vi "C_CAN_Deserialize.vi"(8 "error in (no error)":errorcluster, 11 "payload":u8[](array[numeric]) format="%.0x") -> (0 "error out":errorcluster, 2 "decode errors":u32, 3 "frames":T1[](array[typedef]) {"id" format="%.0x"})   [LabVIEW 2021, in "CANsub_C.lvlib"]
doc: "Decodes all CAN frames of one HDLC payload from the CANsub into CAN_Frame clusters (device time, ID, flags, DLC, data). decode errors = 1 if the payload ended in a truncated frame. Allocates on every call: tests only."
uses:
  CANsub_C.lvlib
  common/Typedefs/Bytes.ctl
  common/CANsub_Common.lvlib
  common/Typedefs/CAN_Frame.ctl
  codec_vis/CANsub_Codec.lvlib
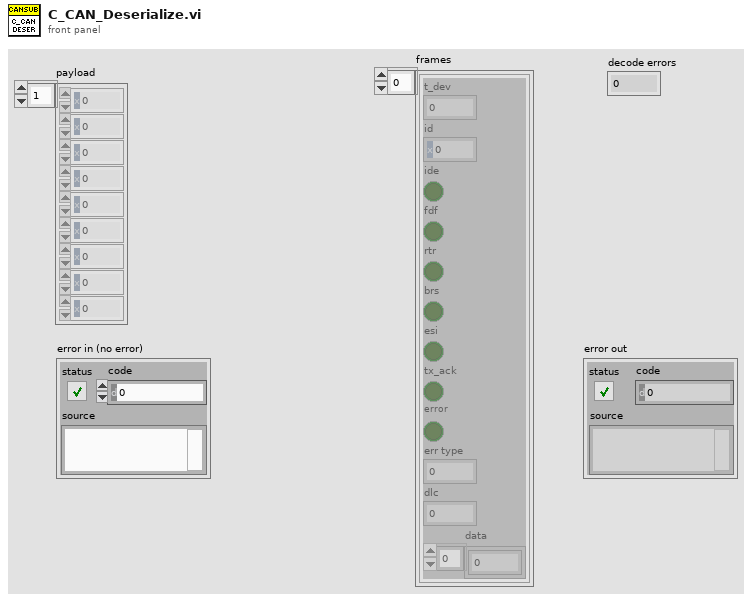
[diagram p1: front panel]
types:
  T1 = typedef "CANsub_Common.lvlib/CAN_Frame.ctl" = cluster{"t_dev":dbl, "id":u32, "ide":bool, "fdf":bool, "rtr":bool, "brs":bool, "esi":bool, "tx_ack":bool, "error":bool, "err type":u8, "dlc":u8, "data":T2}
  T2 = typedef "CANsub_Common.lvlib/Bytes.ctl" = u8[]
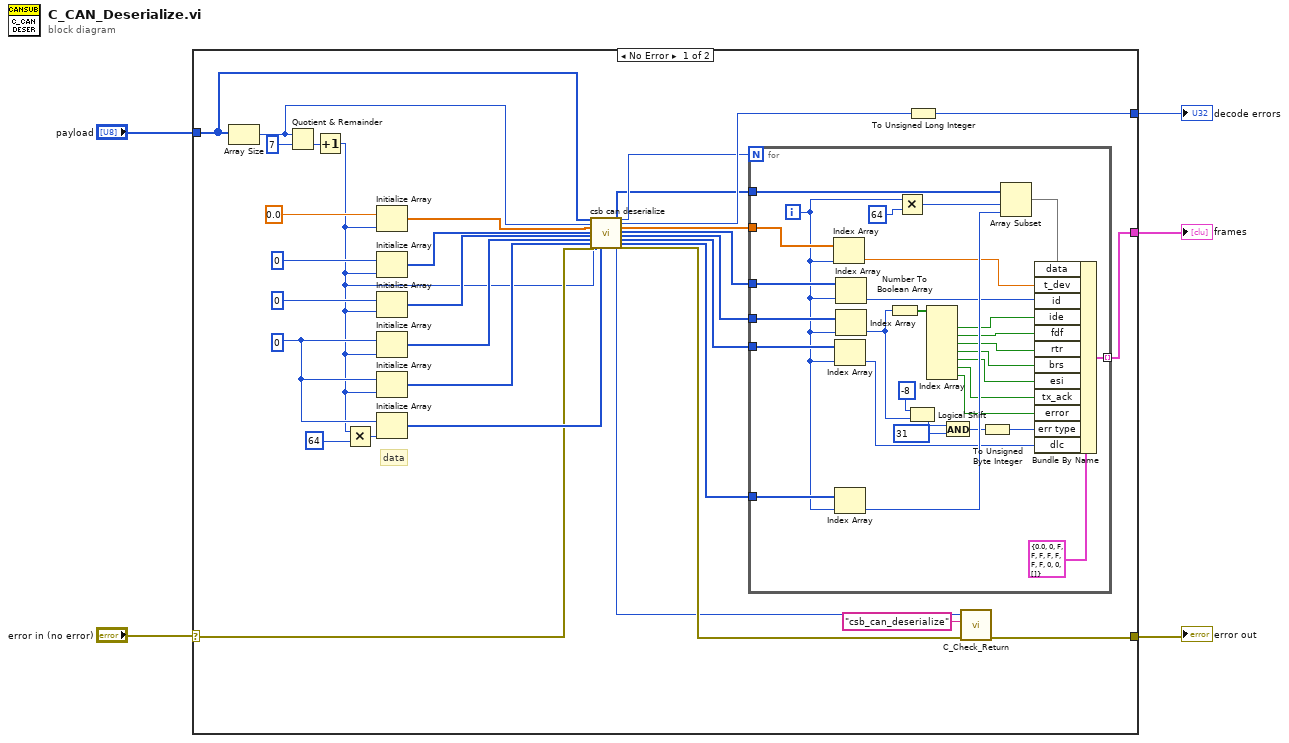
[diagram p0: block diagram]
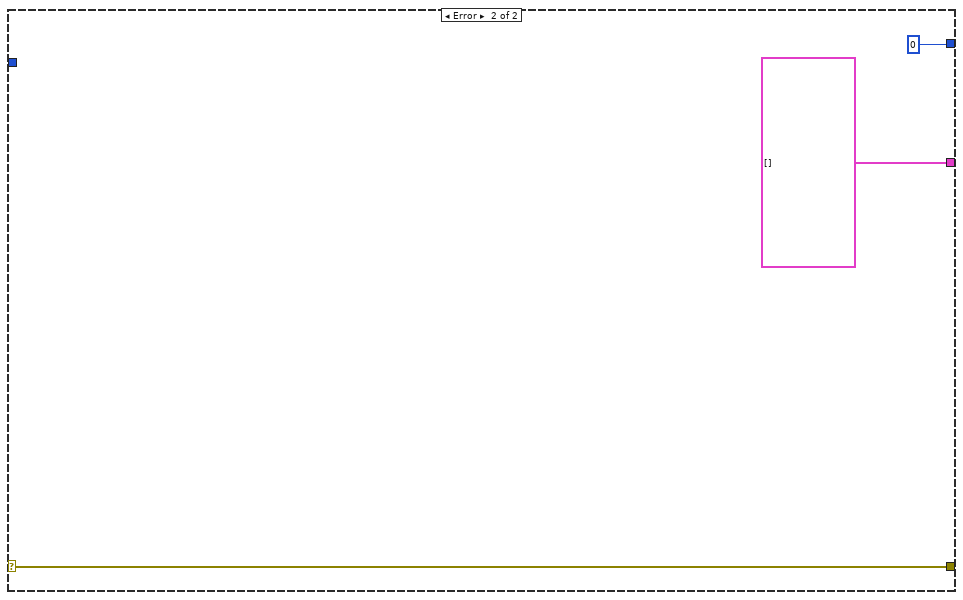
[diagram p2: hidden frame]
diagram:
  n1 = case shown="No Error" "error in (no error)" {
    selector: "error in (no error)" -> [w21 w70]
    tunnel: [w19 w70] -> w4
    tunnel: [w16 u32 0] -> w3
    tunnel: [w6 T1[] [] ("frames")] -> w2
    tunnel: "payload" -> [w28 _]
    frame No Error {
      w36 = u8 0
      # "data"
      n2 = Array Size(array=w28) -> (size(s)=w31:i32)
      n3 = Quotient & Remainder(x=w31, y=7) -> (floor(x/y)=w22:i32)  [unwired: 1 out]
      n4 = Increment(x=w22) -> (x+1=w18:i32)
      n5 = Multiply(x=w18, y=64) -> (x*y=w30:i32)
      n6 = Initialize Array(0.0, w18) -> (w32:dbl[])
      n7 = Initialize Array(u32 0, w18) -> (w23:u32[])
      n8 = Initialize Array(u16 0, w18) -> (w24:u16[])
      n9 = Initialize Array(w36, w18) -> (w25:u8[])
      n10 = Initialize Array(w36, w18) -> (w26:u8[])
      n11 = Initialize Array(w36, w30) -> (w27:u8[])
      n12 = call "csb can deserialize.vi"("payload"=w28, "len"=w31, "t_dev"=w32, "id"=w23, "flags"=w24, "dlc"=w25, "data_len"=w26, "error in (no error)"=w21, "max_frames"=w18, "data"=w27) -> ("data out"=w12:u8[], "function return"=w15:i32, "n_frames"=w13:i32, "decode_errors"=w17:i32, "t_dev out"=w11:dbl[], "id out"=w10:u32[], "flags out"=w9:u16[], "dlc out"=w8:u8[], "data_len out"=w7:u8[], "error out"=w20:errorcluster)  [unwired: 8 in]
      n13 = for {
        N: w13 -> [_]
        tunnel: w12 -> [w67]
        tunnel: w11 -> [w66]
        tunnel: w10 -> [w65]
        tunnel: w9 -> [w64]
        tunnel: w8 -> [w63]
        tunnel: w7 -> [w62]
        tunnel: [w53] -> w6 mode=indexing
        i -> [w60]
        n14 = Index Array(array=w66, index=w60) -> (element=w55:dbl)
        n15 = Index Array(array=w63, index=w60) -> (element=w52:u8)
        n16 = Index Array(array=w62, index=w60) -> (element=w61:u8)
        n17 = Index Array(array=w65, index=w60) -> (element=w54:u32)
        n18 = Index Array(array=w64, index=w60) -> (element=w43:u16)
        n19 = Number To Boolean Array(number=w43) -> (Boolean array=w51:bool[])
        n20 = Multiply(x=w60, y=64) -> (x*y=w58:i32)
        n21 = Logical Shift(y=i16 -8, x=w43) -> (x << y=w41:u16)
        n22 = Index Array(array=w51) -> (element #1=w50:bool, element #2=w49:bool, element #3=w48:bool, element #4=w47:bool, element #5=w46:bool, element #6=w45:bool, element #7=w44:bool)  [unwired: 7 in]
        n23 = And(x=w41, y=u16 31) -> (x .and. y?=w39:u16)
        n24 = To Unsigned Byte Integer(number=w39) -> (unsigned 8bit integer=w38:u8)
        n25 = Array Subset(array=w67, index=w58, length=w61) -> (w56:u8[])
        n26 = Bundle By Name(cluster=T1 {"t_dev"=0.0, "id"=0, "ide"=FALSE, "fdf"=FALSE, "rtr"=FALSE, "brs"=FALSE, "esi"=FALSE, "tx_ack"=FALSE, "error"=FALSE, "err type"=0, "dlc"=0, "data"=[]} ("CAN_Frame"), "data"=w56, "t_dev"=w55, "id"=w54, "ide"=w50, "fdf"=w49, "rtr"=w48, "brs"=w47, "esi"=w46, "tx_ack"=w45, "error"=w44, "err type"=w38, "dlc"=w52) -> (w53:T1)
      }
      n27 = To Unsigned Long Integer(number=w17) -> (unsigned 32bit integer=w16:u32)
      n28 = call "C_Check_Return.vi"("error in (no error)"=w20, "function name"="csb_can_deserialize", "function return"=w15) -> ("error out"=w19:errorcluster)  [unwired: 6 in, 2 out]
    }
    frame Error {
    }
  }
  "error out" <- w4
  "frames" <- w2
  "decode errors" <- w3
